vi "RemoteVI Format Duration.vi"(0 "seconds":dbl) -> (4 "text":string)   [LabVIEW 2020, in "RemoteVI.lvlib"]
doc: "Writes a duration in whole seconds (rounded down, negative counts as 0) as 12 s, 3 min 5 s or 2 h 7 min - for the status text (RemoteVI Status Text.vi). Pure function, cannot fail. Reference: formatDuration() in tools\\lib\\status.mjs, vectors tests\\vectors\\status.json (durations)."
uses:
  RemoteVI.lvlib
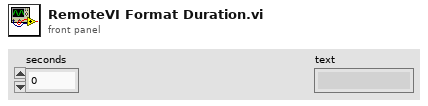
[diagram p1: front panel]
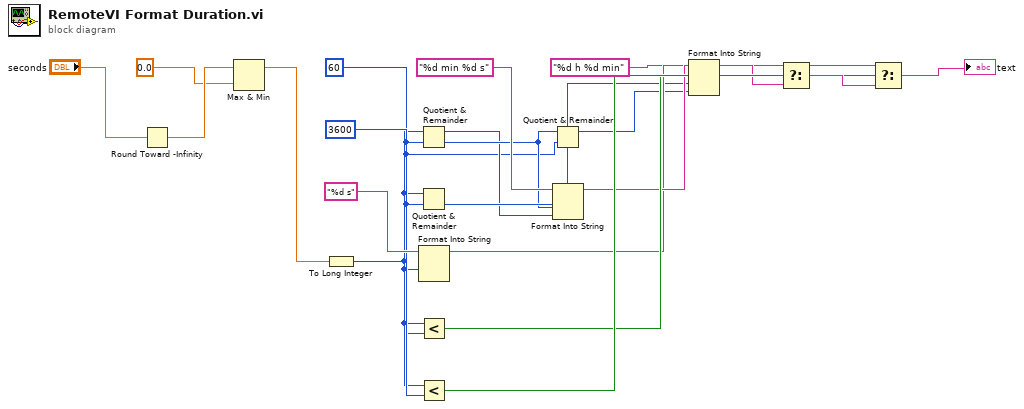
[diagram p0: block diagram]
diagram:
  w7 = 3600
  w6 = 60
  n1 = Round Toward -Infinity(1:"seconds") -> (0:w3:dbl)
  n2 = Max & Min(x=w3, y=0.0) -> (max(x,y)=w4:dbl)  [unwired: 1 out]
  n3 = To Long Integer(number=w4) -> (32bit integer=w5:i32)
  n4 = Quotient & Remainder(x=w5, y=w6) -> (x-y*floor(x/y)=w8:i32, floor(x/y)=w9:i32)
  n5 = Quotient & Remainder(x=w5, y=w7) -> (floor(x/y)=w10:i32)  [unwired: 1 out]
  n6 = Format Into String(format string="%d s", w5) -> (resulting string=w15:string)  [unwired: 2 in, 1 out]
  n7 = Less?(x=w5, y=w6) -> (x < y?=w18:bool)
  n8 = Less?(x=w5, y=w7) -> (x < y?=w19:bool)
  n9 = Quotient & Remainder(x=w9, y=w6) -> (x-y*floor(x/y)=w11:i32)  [unwired: 1 out]
  n10 = Format Into String(format string="%d min %d s", w9, w8) -> (resulting string=w16:string)  [unwired: 2 in, 1 out]
  n11 = Format Into String(format string="%d h %d min", w10, w11) -> (resulting string=w17:string)  [unwired: 2 in, 1 out]
  n12 = Select(t=w16, s=w19, f=w17) -> (s? t:f=w20:string)
  n13 = Select(t=w15, s=w18, f=w20) -> (s? t:f=→"text":string)
